vi "Process Container.vi"() -> ()   [LabVIEW 2020, in "Caraya.lvlib" / "Basic Test Manager.lvclass"]
uses:
  Basic Test Manager.lvclass
  Test Manager Message/TestManagerMsg.lvclass
panel:
  out "error":errorcluster
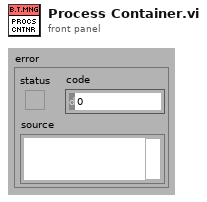
[diagram p1: front panel]
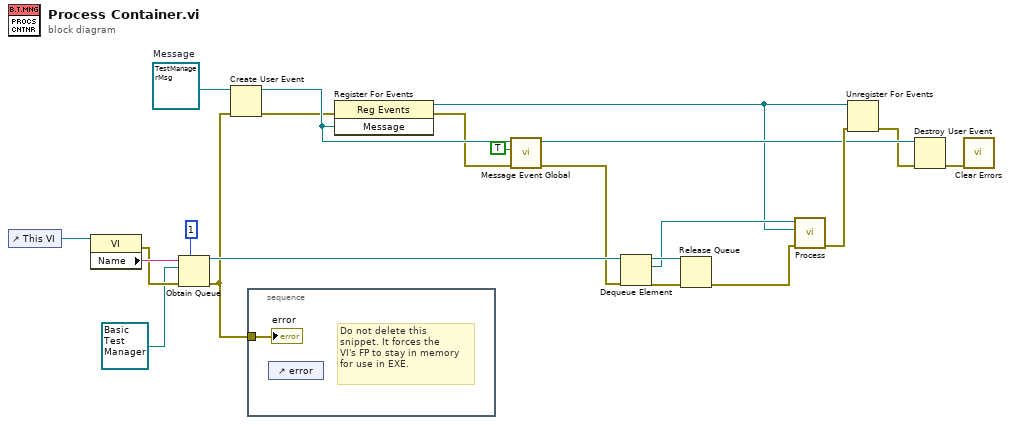
[diagram p0: block diagram]
diagram:
  w11 = refnum<class "TestManagerMsg.lvclass"> refnum  # Message
  n1 = control-ref of="This VI"() -> (w22:refnum<vi>)
  n2 = property class="VI"(reference=w22) -> (error out=w20:errorcluster, "Name"=w21:string)  [unwired: 1 in, 1 out]
  n3 = Obtain Queue(max queue size (-1, unlimited)=1, name (unnamed)=w21, element data type=refnum<class "Basic Test Manager.lvclass"> refnum ("element"), error in (no error)=w20) -> (queue out=w17:refnum<queue>, error out=w10:errorcluster)  [unwired: 1 in, 1 out]
  n4 = Create User Event(user event datatype=w11, error in=w10) -> (user event=w9:refnum<user-event>, error out=w2:errorcluster)
  n5 = stacked-sequence {
    tunnel: w10 -> [w23]
    frame #0 {
      # "Do not delete this\nsnippet. It forces the\nVI's FP to stay in memory\nfor use in EXE."
      n6 = control-ref of="error"() -> ()  [unwired: 1 out]
      "error" <- w23
    }
  }
  n7 = register-events(error in=w2, w9) -> (reference out=w1:refnum<event-registration>, error out=w8:errorcluster)  [unwired: 1 in]
  n8 = call "Message Event Global.vi"("error in (no error)"=w8, "Set (F)"=TRUE, "Message Event in"=w9) -> ("error out"=w3:errorcluster, "Message Event out"=w6:refnum<user-event>)  [unwired: 5 in, 2 out]
  n9 = Dequeue Element(queue=w17, error in (no error)=w3) -> (queue out=w16:refnum<queue>, element=w14:refnum<class "Basic Test Manager.lvclass">, error out=w15:errorcluster)  [unwired: 1 in, 1 out]
  n10 = Release Queue(queue=w16, error in (no error)=w15) -> (error out=w13:errorcluster)  [unwired: 1 in, 2 out]
  n11 = call "Process.vi"("error in (no error)"=w13, "Event Registration Refnum"=w1, "Test Manager"=w14) -> ("error out"=w12:errorcluster)  [unwired: 7 in, 1 out]
  n12 = Unregister For Events(event registration refnum=w1, error in=w12) -> (error out=w4:errorcluster)
  n13 = Destroy User Event(user event=w6, error in=w4) -> (error out=w5:errorcluster)
  n14 = call <vilib>:"Clear Errors.vi"("error in (no error)"=w5) -> ()  [unwired: 5 in, 2 out]
